vi "WLAN Fetch TxP.vi"(0 "Instrument Handle In":refnum<k21>, 1 "Selector String":string, 11 "error in (no error)":errorcluster) -> (4 "Instrument Handle Out":refnum<k21>, 6 "TxP Results":T1 {"Average Power Mean (dBm)" format="%.2f"; "Peak Power Maximum (dBm)" format="%.2f"}, 15 "error out":errorcluster)   [LabVIEW 2016, in "RFmxWLAN.lvlib"]
doc: "Fetches common results from the TxP measurement."
uses:
  RFmxWLAN.lvlib
  Typedefs/WLAN TxP Results.ctl
  <vilib>/RFmx/WLAN/mx/RFmxWLAN.llb/RFmxWLAN TXP Fetch Measurement.vi
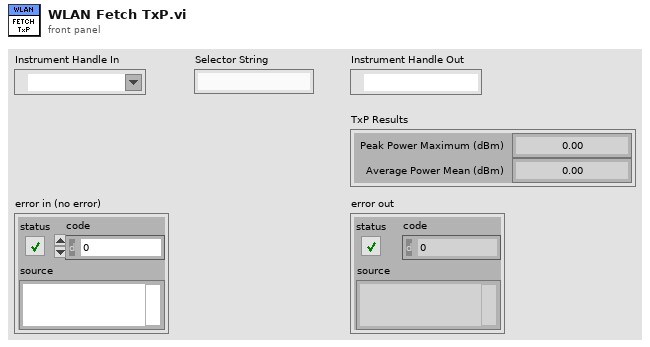
[diagram p1: front panel]
types:
  T1 = typedef "RFmxWLAN.lvlib/WLAN TxP Results.ctl" = cluster{"Peak Power Maximum (dBm)":dbl, "Average Power Mean (dBm)":dbl}
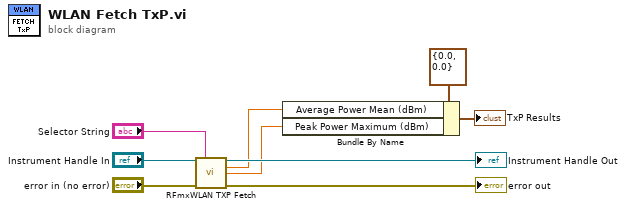
[diagram p0: block diagram]
diagram:
  n1 = call-poly <vilib>:"RFmxWLAN TXP Fetch.vi"("Instrument Handle In"="Instrument Handle In", "Selector String"="Selector String", "error in (no error)"="error in (no error)") -> ("Instrument Handle Out"=→"Instrument Handle Out":refnum<k21>, "Average Power Mean (dBm)"=w2:dbl, "Peak Power Maximum (dBm)"=w1:dbl, "error out"=→"error out":errorcluster)  [unwired: 9 in]
  n2 = Bundle By Name(cluster=T1 {"Peak Power Maximum (dBm)"=0.0, "Average Power Mean (dBm)"=0.0} ("WLAN TxP Results"), "Average Power Mean (dBm)"=w2, "Peak Power Maximum (dBm)"=w1) -> (→"TxP Results":T1)
